vi "Run.vi"(8 "error in":errorcluster) -> (0 "error out":errorcluster)   [LabVIEW 2024]
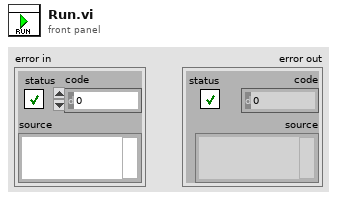
[diagram p1: front panel]
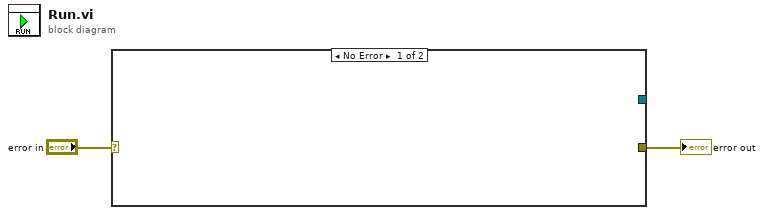
[diagram p0: block diagram]
diagram:
  n1 = case shown="No Error" "error in" {
    selector: "error in" -> [_ w4]
    tunnel: [_ w4] -> w1
    tunnel: _ -> [_ w3]
    frame No Error {
    }
    frame Error {
    }
  }
  "error out" <- w1
